vi "Enqueue File.vi"(10 "filepath":path, 11 "Blocks queue":refnum<queue>) -> (2 "error out":errorcluster)   [LabVIEW 2013, in "MD5.lvlib" / "MD5.lvclass"]
uses:
  MD5.lvclass
  Data-vector.ctl
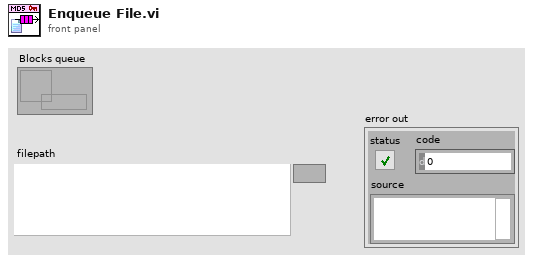
[diagram p1: front panel]
types:
  T1 = enum16{"open", "replace", "create", "open or create", "replace or create", "replace or create with confirmation"}
  T2 = typedef "MD5.lvlib/MD5.lvclass/Data-vector.ctl" = cluster{"Data[ ]":u8[], "end":bool}
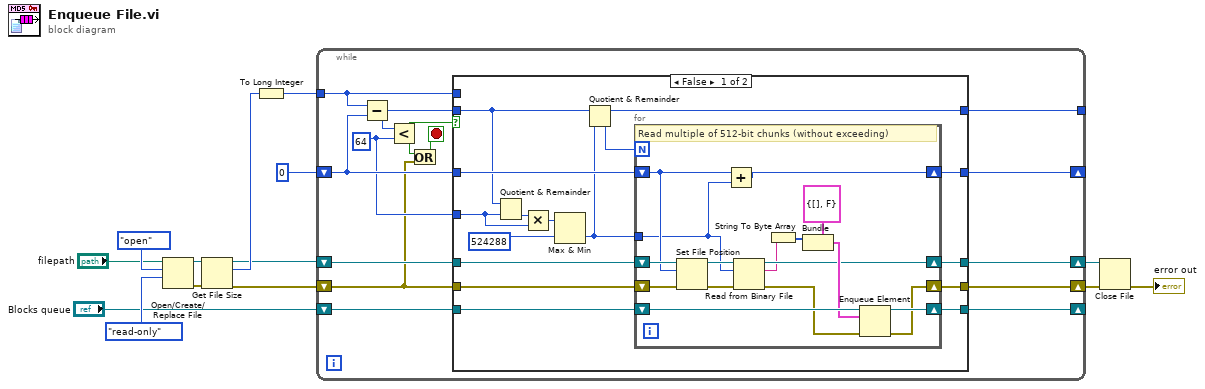
[diagram p0: block diagram]
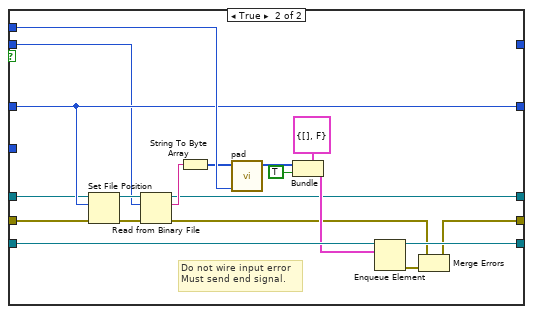
[diagram p2: hidden frame]
diagram:
  n1 = Open/Create/Replace File(file path (use dialog)="filepath", operation (0:open)=T1."open", access (0:read/write)=enum16{"read/write", "read-only", "write-only"}."read-only") -> (refnum out=w13:refnum<file>, error out=w12:errorcluster)  [unwired: 3 in, 1 out]
  n2 = Get File Size(file=w13, error in=w12) -> (refnum out=w5:refnum<file>, size (in bytes)=w8:i64, 0:w4:errorcluster)
  n3 = To Long Integer(number=w8) -> (32bit integer=w7:i32)
  n4 = while {
    shift-right: [w24] -> _
    shift-left: 0 ("offset") -> [w26]
    tunnel: w7 -> [w20]
    tunnel: [w25] -> _
    shift-right: [w27] -> _
    shift-left: "Blocks queue" -> [w28]
    shift-right: [w19] -> w3
    shift-left: w5 -> [w23]
    shift-right: [w18] -> w2
    shift-left: w4 -> [w17]
    stop <- w15 stop-if-true
    w21 = 64 ("y")
    n5 = Subtract(x=w20, y=w26) -> (x-y=w22:i32)
    n6 = Less?(x=w22, y=w21) -> (x < y?=w16:bool)
    n7 = Or(x=w16, y=w17) -> (x .or. y?=w15:bool)
    n8 = case shown="False" w16 {
      tunnel: w28 -> [w44 w78]
      tunnel: [w43 w77] -> w27
      tunnel: w26 -> [w42 w72]
      tunnel: [w36 _] -> w25
      tunnel: [w35 w72] -> w24
      tunnel: w23 -> [w34 w71]
      tunnel: w22 -> [w33 w66]
      tunnel: w21 -> [w32 _]
      tunnel: w20 -> [_ w79]
      tunnel: [w31 w65] -> w19
      tunnel: w17 -> [w30 w64]
      tunnel: [w29 w61] -> w18
      frame False {
        n9 = Quotient & Remainder(x=w33, y=w32) -> (floor(x/y)=w41:i32)  [unwired: 1 out]
        n10 = Multiply(x=w41, y=w32) -> (x*y=w40:i32)
        n11 = Max & Min(x=w40, y=524288) -> (min(x,y)=w37:i32)  [unwired: 1 out]
        n12 = Quotient & Remainder(x=w33, y=w37) -> (x-y*floor(x/y)=w36:i32, floor(x/y)=w38:i32)
        n13 = for {
          N: w38 -> [_]
          shift-right: [w59] -> w43
          shift-left: w44 -> [w60]
          shift-right: [w56] -> w35
          shift-left: w42 -> [w53]
          tunnel: w37 -> [w51]
          shift-right: [w50] -> w31
          shift-left: w34 -> [w55]
          shift-right: [w45] -> w29
          shift-left: w30 -> [w48]
          # "Read multiple of 512-bit chunks (without exceeding)"
          n14 = Set File Position(offset (in bytes) (0)=w53, refnum=w55, error in=w48) -> (refnum out=w52:refnum<file>, error out=w47:errorcluster)  [unwired: 1 in]
          n15 = Add(x=w53, y=w51) -> (x+y=w56:i32)
          n16 = Read from Binary File(8:w47, 10:w51, 11:w52) -> (0:w46:errorcluster, 2:w49:string, 3:w50:refnum<file>)  [unwired: 3 in, 1 out]
          n17 = String To Byte Array(string=w49) -> (unsigned byte array=w54:u8[])
          n18 = Bundle(cluster=T2 {"Data[ ]"=[], "end"=FALSE}, "Data[ ]"=w54) -> (w57:T2)  [unwired: 1 in]
          n19 = Enqueue Element(queue=w60, element=w57, error in (no error)=w46) -> (queue out=w59:refnum<queue>, error out=w45:errorcluster)  [unwired: 1 in, 1 out]
        }
      }
      frame True {
        # "Do not wire input error\nMust send end signal."
        n20 = Set File Position(offset (in bytes) (0)=w72, refnum=w71, error in=w64) -> (refnum out=w69:refnum<file>, error out=w70:errorcluster)  [unwired: 1 in]
        n21 = Read from Binary File(8:w70, 10:w66, 11:w69) -> (0:w62:errorcluster, 2:w68:string, 3:w65:refnum<file>)  [unwired: 3 in, 1 out]
        n22 = String To Byte Array(string=w68) -> (unsigned byte array=w67:u8[])
        n23 = call "pad.vi"("data length"=w79, "Last Block"=w67) -> ("Padding"=w75:u8[])  [unwired: 8 in, 1 out]
        n24 = Bundle(cluster=T2 {"Data[ ]"=[], "end"=FALSE}, "Data[ ]"=w75, "end"=TRUE) -> (w73:T2)
        n25 = Enqueue Element(queue=w78, element=w73) -> (queue out=w77:refnum<queue>, error out=w63:errorcluster)  [unwired: 2 in, 1 out]
        n26 = Merge Errors(w62, w63) -> (w61:errorcluster)
      }
    }
  }
  n27 = Close File(refnum=w3, error in=w2) -> (error out=→"error out":errorcluster)  [unwired: 1 out]
